vi "SC Deploy Dialog.vi"(8 "changes?":bool=TRUE, 9 "project":string, 10 "robot":string, 11 "add-ons":string[](array[string])) -> (1 "message":string, 2 "deploy?":bool)   [LabVIEW 2023]
doc: "Before a deploy: shows the project, robot and add-ons, asks for an optional description of the change (the commit message for uncommitted changes), and returns deploy? = false when the user cancels or closes the window."
uses:
  <vilib>/Utility/error.llb/Trim Whitespace One-Sided.vi
panel:
  in  "Cancel":bool
  in  "Deploy":bool
  in  "Describe the change (optional)":string
  out "Summary":string
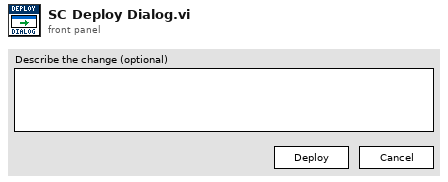
[diagram p1: front panel]
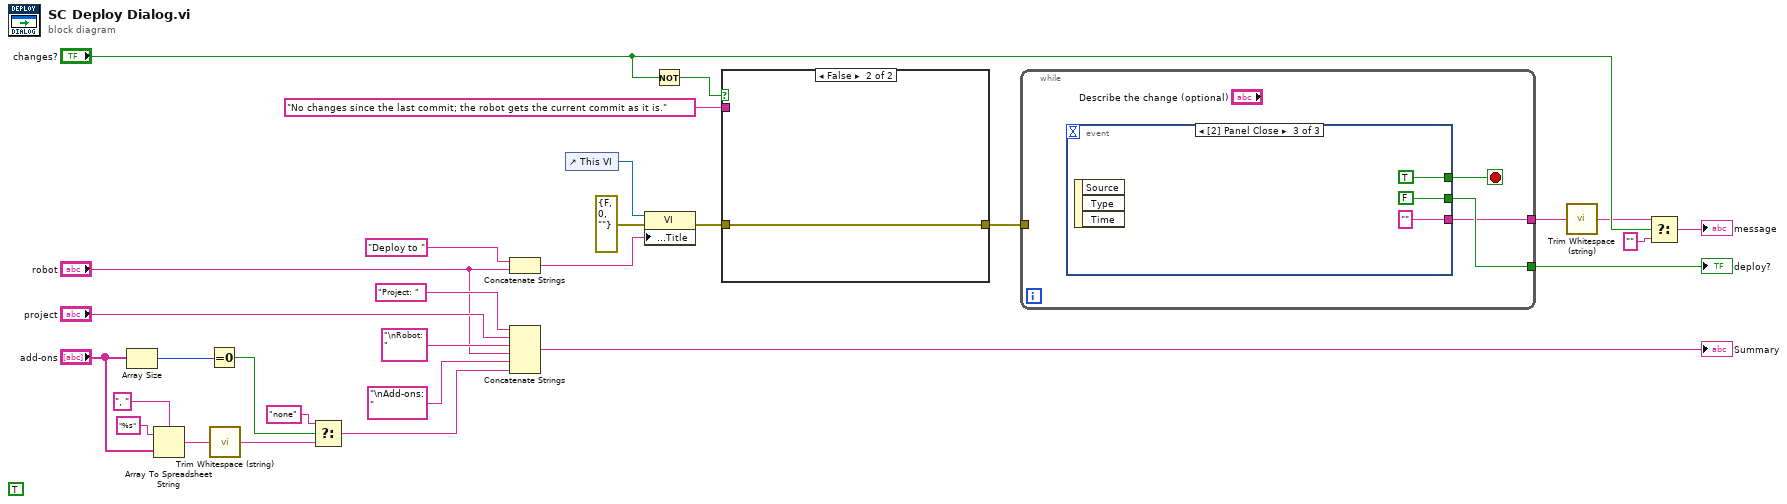
[diagram p0: block diagram]
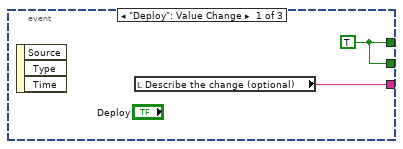
[diagram p2: hidden frame]
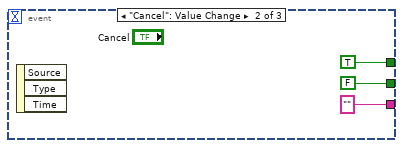
[diagram p3: hidden frame]
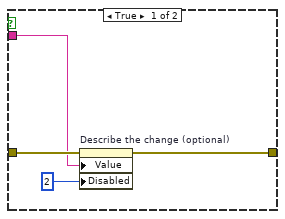
[diagram p4: hidden frame]
diagram:
  (unwired) TRUE
  n1 = Array Size(array="add-ons") -> (size(s)=w25:i32)
  n2 = Array To Spreadsheet String(delimiter (Tab)=", ", array="add-ons", 3:"%s") -> (spreadsheet string=w27:string)
  n3 = Equal To 0?(x=w25) -> (x = 0?=w24:bool)
  n4 = call <vilib>:"Trim Whitespace (string).vi"("string"=w27) -> ("trimmed string"=w22:string)  [unwired: 1 in]
  n5 = Select(t="none", s=w24, f=w22) -> (s? t:f=w17:string)
  n6 = Concatenate Strings("Deploy to ", "robot") -> (w11:string)
  n7 = Concatenate Strings("Project: ", "project", "\nRobot: ", "robot", "\nAdd-ons: ", w17) -> (→"Summary":string)
  n8 = control-ref of="This VI"() -> (w13:refnum<vi>)
  n9 = property class="VI"(reference=w13, error in=errorcluster {"status"=FALSE, "code"=0, "source"=""}, "Front Panel Window:Title"=w11) -> (error out=w9:errorcluster)  [unwired: 1 out]
  n10 = Not(x="changes?") -> (.not. x?=w8:bool)
  n11 = case shown="False" w8 {
    tunnel: "No changes since the last commit; the robot gets the current commit as it is." -> [w32 _]
    tunnel: w9 -> [w33 w34]
    tunnel: [w30 w34] -> w7
    frame True {
      n12 = property on="Describe the change (optional)" class="Str"(error in=w33, "Value"=w32, "Disabled"=u8 2) -> (error out=w30:errorcluster)  [unwired: 1 in, 1 out]
    }
    frame False {
    }
  }
  n13 = while {
    tunnel: w7 -> [_]
    tunnel: [w36] -> w6
    tunnel: [w35] -> w5
    stop <- w37 stop-if-true
    n14 = event shown="[2] Panel Close" {
      selector: _ -> [_ _ _]
      dyn-events: _ -> [_ _ _]
      timeout: _ -> [_ _ _]
      tunnel: [w39 TRUE TRUE] -> w37
      tunnel: [w39 FALSE FALSE] -> w36
      tunnel: [w38 "" ""] -> w35
      event "Deploy": Value Change {
        w39 = TRUE
        n15 = event-data() -> ()  [unwired: 1 in, 3 out]
        n16 = local read "Describe the change (optional)"() -> (w38:string)
      }
      event "Cancel": Value Change {
        n17 = event-data() -> ()  [unwired: 1 in, 3 out]
      }
      event Panel Close {
        n18 = event-data() -> ()  [unwired: 1 in, 3 out]
      }
    }
  }
  "deploy?" <- w6
  n19 = call <vilib>:"Trim Whitespace (string).vi"("string"=w5) -> ("trimmed string"=w3:string)  [unwired: 1 in]
  n20 = Select(t=w3, s="changes?", f="") -> (s? t:f=→"message":string)
